vi "OwnCompat20261012_Native_GetDiagramObjects.vi"() -> ()   [LabVIEW 2024]
panel:
  out "error out":errorcluster caption="错误输出"
  out "object_ids":u32[](array[numeric])
  in  "object_ids type":u32
  in  "diagram_id":u32
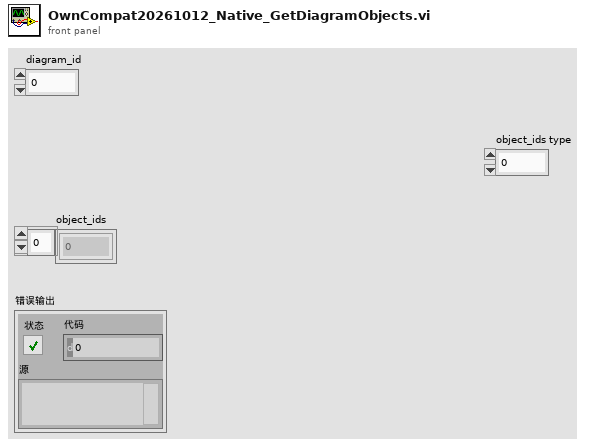
[diagram p1: front panel]
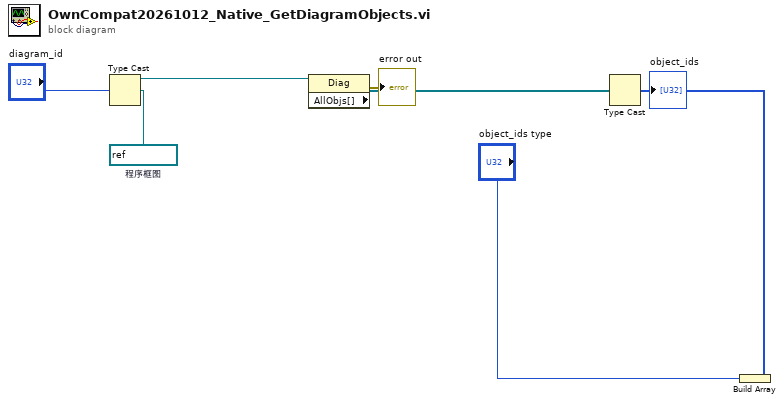
[diagram p0: block diagram]
diagram:
  w7 = refnum<vi> refnum  # 程序框图
  n1 = Type Cast ("强制类型转换")(type=w7, x="diagram_id") -> (*(type *) &x=w6:refnum<vi>)
  n2 = property on="属性节点" class="Diag"(reference=w6) -> (error out=→"error out":errorcluster, "AllObjs[]"=w5:refnum<vi>[])  [unwired: 1 in, 1 out]
  n3 = Build Array ("创建数组")("object_ids type") -> (w3:u32[])
  n4 = Type Cast ("强制类型转换")(type=w3, x=w5) -> (*(type *) &x=→"object_ids":u32[])
